vi "Disable Control.vi"(8 "error in (no error)":errorcluster, 9 "Disabled":T1(ring), 10 "FP Item Name":string, 11 "Father of all uServices in":refnum<class "Father of all uServices.lvclass">) -> (0 "error out":errorcluster, 3 "Father of all uServices out":refnum<class "Father of all uServices.lvclass">)   [LabVIEW 2020, in "TALOS.lvlib" / "Father of all uServices.lvlib" / "Father of all uServices.lvclass"]
uses:
  Father of all uServices.lvclass
  Ancestor/Ancestor/Ancestor.lvclass/Ancestor.ctl
  Support VIs/Generate Error.vi
  FGV/Error Memory/Get Error Description.vi
  Support VIs/Get PC name.vi
  Ancestor/Ancestor/Read ID.vi
  Support VIs/Get Class Name.vi
  <vilib>/Utility/error.llb/Clear Errors.vi
  FGV/Error Memory/Error Memory Core.vi
  <vilib>/AdvancedString/Delimited String to 1D String Array.vi
  Support VIs/Circus Root Path.vi
  FGV/Error Memory/Error Crt Lvl checker.vi
  FGV/Error Memory/Error Memory Core.vi/40c8088d-b597-4017-91af-faa98e00292e.vi
  FGV/Error Memory/Error Memory Core.vi/d4a3ab98-063c-4e44-b43d-fbdcfe6c2be2.vi
  Support VIs/Global Memory.vi
  <vilib>/Utility/LVClass/Get LV Class Name.vi
  Support VIs/Is in Packed Library.vi
  Support VIs/TALOS Root path.vi
  Support VIs/Read CSV worksheet.vi
  Support VIs/Global Constants.vi
  <vilib>/Utility/error.llb/General Error Handler.vi
  Support VIs/Error Log.vi
  Ancestor/Ancestor/Ancestor.lvclass
  <vilib>/Comparison/Equal/Equal Functor/Equal Functor.lvclass
  TALOS.lvlib
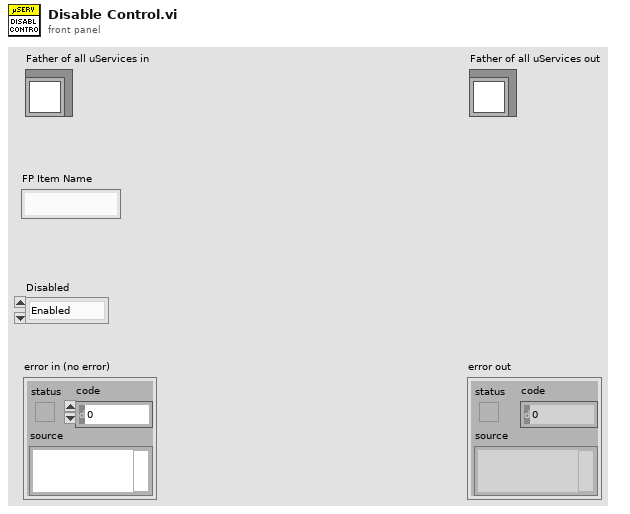
[diagram p1: front panel]
types:
  T1 = enum8{"Enabled", "Disabled", "Disabled and Grayed Out"}
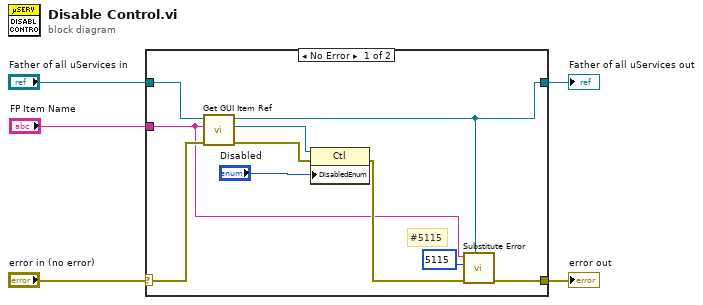
[diagram p0: block diagram]
diagram:
  n1 = case shown="No Error" "error in (no error)" {
    selector: "error in (no error)" -> [w14 w17]
    tunnel: [w13 w17] -> w4
    tunnel: [w6 w16] -> w2
    tunnel: "Father of all uServices in" -> [w11 w16]
    tunnel: "FP Item Name" -> [w8 _]
    frame No Error {
      # "#5115"
      n2 = call "Get GUI Item Ref.vi"("error in (no error)"=w14, "FP Item Name"=w8, "uService Template in"=w11) -> ("error out"=w10:errorcluster, "Ctl Refnum"=w15:refnum<vi>, "uService Template out"=w6:refnum<class "Father of all uServices.lvclass">)  [unwired: 6 in]
      n3 = property class="Ctl"(reference=w15, error in=w10, "DisabledEnum"="Disabled") -> (error out=w12:errorcluster)  [unwired: 1 out]
      n4 = call "Substitute Error.vi"("LabVIEW Object"=w6, "error in (no error)"=w12, "Error Code"=5115, "Optional String"=w8) -> ("error out"=w13:errorcluster)  [unwired: 7 in]
    }
    frame Error {
    }
  }
  "error out" <- w4
  "Father of all uServices out" <- w2
